vi "uRedRTP.vi"() -> ()   [LabVIEW 2019]
uses:
  <vilib>/FPGAPlugInAG/myRIO-1900/niLvFpga_Open_myRIO-1900.vi
  <vilib>/rvi/interface/common/dynamic/niFpgaDynamicAddResources.vi
  <vilib>/Utility/error.llb/Error Cluster From Error Code.vi
  <vilib>/rvi/errors/niLvFpgaAdjustHostInterfaceError.vi
  <vilib>/FPGAPlugInAG/Dynamic/niLvFpga_Close_Dynamic.vi
  <vilib>/rvi/interface/nirviOpenFPGA/nirviOpenFPGA.xnode
  FPGA Bitfiles/sec_FPGATarget2_uRedFPGA_nmZ84bOtljk.lvbitx
  uRedFPGA.vi
  <vilib>/rvi/interface/nirviReadWriteControl/nirviReadWriteControl.xnode
  <vilib>/rvi/interface/nirviCloseFPGA/nirviCloseFPGA.xnode
  NiFpgaLv.dll
  <vilib>/rvi/interface/Simulation/niFpgaSimulationCallBeginRW.vi
panel:
  out "SoCMin":bool
  out "BlocIb":bool
  out "Ib_Out":i16
  out "Vg":bool
  out "PL>PPV":bool
  out "SoC<0.8":bool
  out "mSoC":fxp<+/-,64,4>
  out "ib":fxp<+/-,64,31>
  out "Time":u32
  out "SoC":dbl(graph)
  out "Potencias":cluster{dbl, dbl, dbl}(graph)
  in  "stop":bool
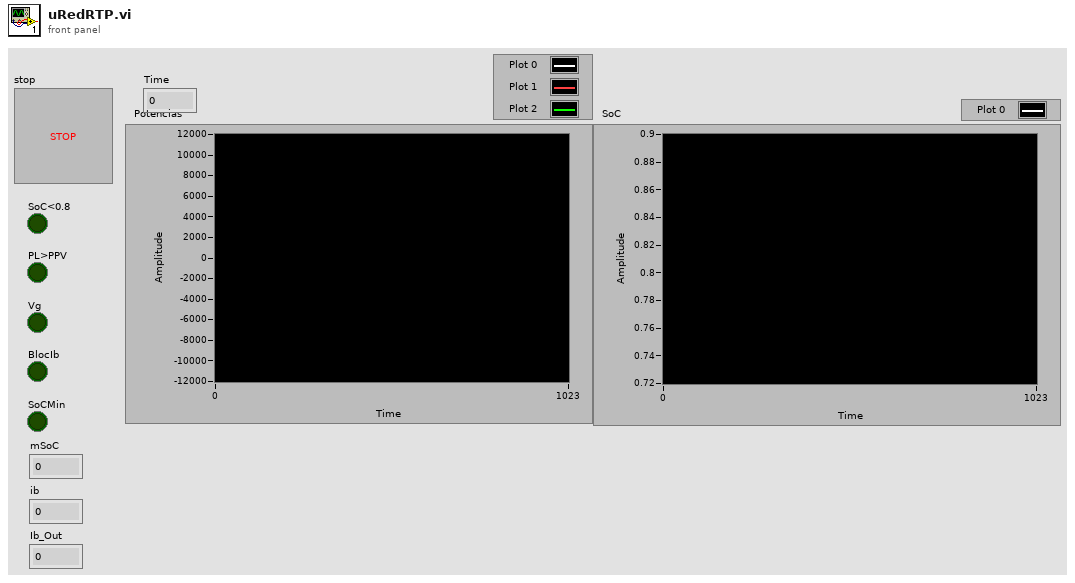
[diagram p1: front panel]
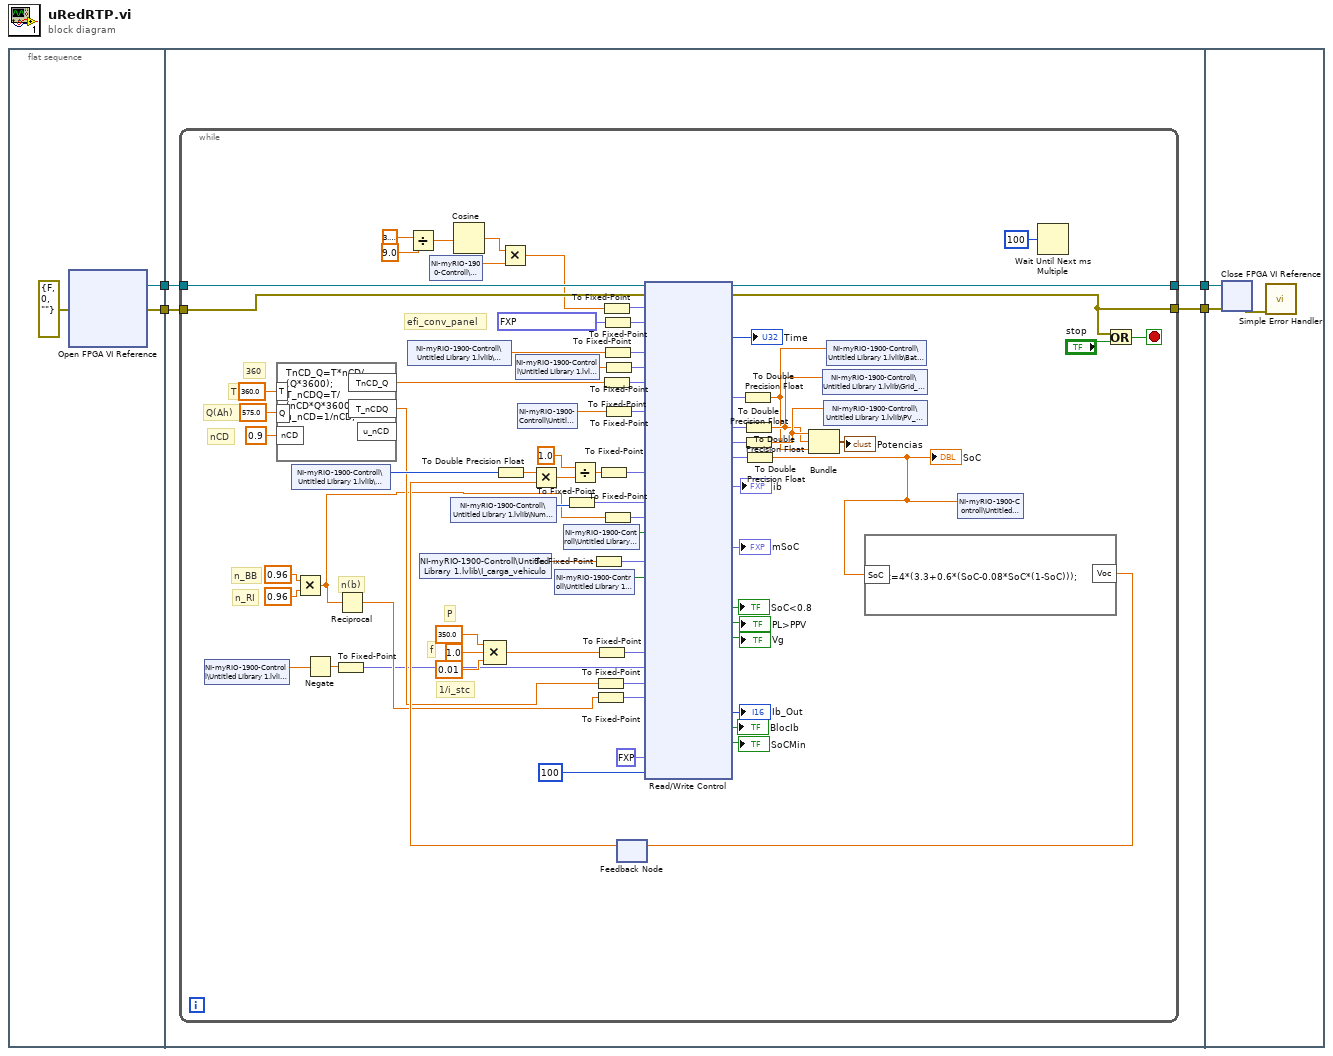
[diagram p0: block diagram]
diagram:
  n1 = flat-sequence {
    tunnel: [w7] -> w4
    tunnel: [w6] -> w3
    tunnel: w4 -> [w11]
    tunnel: w3 -> [w10]
    tunnel: [w9] -> w2
    tunnel: [w8] -> w1
    tunnel: w2 -> [w91]
    tunnel: w1 -> [w90]
    frame #0 {
      n2 = xnode "Open FPGA VI Reference"("error in"=errorcluster {"status"=FALSE, "code"=0, "source"=""}) -> ("FPGA VI Reference Out"=w7:refnum<k20>, "error out"=w6:errorcluster)  [unwired: 1 in]
    }
    frame #1 {
      n3 = while {
        tunnel: w11 -> [w86]
        tunnel: w10 -> [w85]
        tunnel: [w84] -> w9
        tunnel: [w83] -> w8
        stop <- w88 stop-if-true
        # "360"
        # "efi_conv_panel"
        # "n(b)"
        # "n_RI"
        # "n_BB"
        # "1/i_stc"
        # "f"
        # "P"
        # "nCD"
        # "T"
        # "Q(Ah)"
        n4 = shared-variable "NI-myRIO-1900-Controll\\Untitled Library 1.lvlib\\Qch_EV"() -> (w19:dbl)  [unwired: 1 in, 1 out]
        n5 = formula code="TnCD_Q=T*nCD/(Q*3600);\nT_nCDQ=T/(nCD*Q*3600);\nu_nCD=1/nCD;"("T"=360.0 ("x"), "nCD"=0.9 ("y"), "Q"=575.0) -> ("TnCD_Q"=w27:dbl, "T_nCDQ"=w25:dbl)  [unwired: 1 out]
        n6 = shared-variable "NI-myRIO-1900-Controll\\Untitled Library 1.lvlib\\Num_Bats"() -> (w45:u8)  [unwired: 1 in, 1 out]
        n7 = Multiply(x=0.96, y=0.96) -> (x*y=w20:dbl)
        n8 = Negate(x=w19) -> (-x=w18:dbl)
        n9 = To Fixed-Point(number=w18) -> (fixed-point=w17:fxp<+/-,32,16>)  [unwired: 1 in]
        n10 = Reciprocal(x=w20) -> (1/x=w22:dbl)
        n11 = Divide(x=3.141592653589793, y=9.0) -> (x/y=w51:dbl)
        n12 = shared-variable "NI-myRIO-1900-Controll\\Untitled Library 1.lvlib\\LoadPower"() -> (w42:dbl)  [unwired: 1 in, 1 out]
        n13 = shared-variable "NI-myRIO-1900-Controll\\Untitled Library 1.lvlib\\I_carga_vehiculo"() -> (w39:dbl)  [unwired: 1 in, 1 out]
        n14 = shared-variable "NI-myRIO-1900-Controll\\Untitled Library 1.lvlib\\G"() -> (w50:dbl)  [unwired: 1 in, 1 out]
        n15 = shared-variable "NI-myRIO-1900-Controll\\Untitled Library 1.lvlib\\Num_Panel"() -> (w70:u8)  [unwired: 1 in, 1 out]
        n16 = Cosine(x=w51) -> (cos(x)=w49:dbl)
        n17 = Compound Arithmetic op=MULTIPLY(350.0 ("value"), 1.0 ("value"), 0.01 ("value")) -> (w38:dbl)
        n18 = To Double Precision Float(number=w45) -> (double precision float=w46:dbl)
        n19 = Multiply(x=w49, y=w50) -> (x*y=w48:dbl)
        n20 = shared-variable "NI-myRIO-1900-Controll\\Untitled Library 1.lvlib\\SoC_ini"() -> (w69:dbl)  [unwired: 1 in, 1 out]
        n21 = shared-variable "NI-myRIO-1900-Controll\\Untitled Library 1.lvlib\\VG"() -> (w75:dbl)  [unwired: 1 in, 1 out]
        n22 = shared-variable "NI-myRIO-1900-Controll\\Untitled Library 1.lvlib\\Cargar"() -> (w41:bool)  [unwired: 1 in, 1 out]
        n23 = shared-variable "NI-myRIO-1900-Controll\\Untitled Library 1.lvlib\\InSoC"() -> (w55:bool)  [unwired: 1 in, 1 out]
        n24 = To Fixed-Point(number=w70) -> (fixed-point=w57:fxp<+,4,4>)  [unwired: 1 in]
        n25 = To Fixed-Point(number=w39) -> (fixed-point=w40:fxp<+,16,0>)  [unwired: 1 in]
        n26 = To Fixed-Point(number=w25) -> (fixed-point=w26:fxp<+,32,2>)  [unwired: 1 in]
        n27 = To Fixed-Point(number=w22) -> (fixed-point=w21:fxp<+,16,0>)  [unwired: 1 in]
        n28 = To Fixed-Point(number=w38) -> (fixed-point=w31:fxp<+,16,0>)  [unwired: 1 in]
        n29 = To Fixed-Point(number=w48) -> (fixed-point=w77:fxp<+,16,14>)  [unwired: 1 in]
        n30 = To Fixed-Point(number=w27) -> (fixed-point=w81:fxp<+,32,2>)  [unwired: 1 in]
        n31 = To Fixed-Point(number=fxp<+,16,0> 0.67999267578125) -> (fixed-point=w78:fxp<+,16,0>)  [unwired: 1 in]
        n32 = To Fixed-Point(number=w42) -> (fixed-point=w79:fxp<+,45,21>)  [unwired: 1 in]
        n33 = To Fixed-Point(number=w20) -> (fixed-point=w56:fxp<+,16,0>)  [unwired: 1 in]
        n34 = To Fixed-Point(number=w69) -> (fixed-point=w80:fxp<+,32,0>)  [unwired: 1 in]
        n35 = To Fixed-Point(number=w75) -> (fixed-point=w59:fxp<+,16,8>)  [unwired: 1 in]
        n36 = feedback #1() -> (w43:dbl)  [unwired: 1 in]
        n37 = Multiply(x=w46, y=w43) -> (x*y=w67:dbl)
        n38 = Divide(x=1.0, y=w67) -> (x/y=w66:dbl)
        n39 = To Fixed-Point(number=w66) -> (fixed-point=w58:fxp<+,16,8>)  [unwired: 1 in]
        n40 = xnode "Read/Write Control"("FPGA VI Reference In"=w86, "error in"=w85, "G"=w77, "n(p)"=w78, "PL"=w79, "SoC_in"=w80, "T*n(CD)/Q"=w81, "VG"=w59, "1/Voc"=w58, "N_Panel"=w57, "nc(b)"=w56, "P_SoC"=w55, "CC_Constant"=w40, "Cargar"=w41, "P*f/i_stc"=w31, "Q"=w17, "T/(n(CD)*Q)"=w26, "1/nc(b)"=w21, "LimSoC"=fxp<+/-,32,16> 1.0, "Time_ms"=u32 100) -> ("FPGA VI Reference Out"=w84:refnum<k20>, "error out"=w83:errorcluster, "Time(ms)"=→"Time":u32, "Pb"=w65:fxp<+/-,47,23>, "PG"=w64:fxp<+/-,47,23>, "PPV"=w63:fxp<+,45,21>, "SoC"=w62:fxp<+,32,0>, "ib"=→"ib":fxp<+/-,64,33>, "mSoC"=→"mSoC":fxp<+/-,64,4>, "SoC<0.8"=→"SoC<0.8":bool, "PL>PPV"=→"PL>PPV":bool, "Vg"=→"Vg":bool, "Ib_Out"=→"Ib_Out":i16, "BlocIb"=→"BlocIb":bool, "SoCMin"=→"SoCMin":bool)  [unwired: 1 out]
        n41 = To Double Precision Float(number=w65) -> (double precision float=w72:dbl)
        n42 = To Double Precision Float(number=w64) -> (double precision float=w73:dbl)
        n43 = To Double Precision Float(number=w63) -> (double precision float=w74:dbl)
        n44 = To Double Precision Float(number=w62) -> (double precision float=w47:dbl)
        "SoC" <- w47
        n45 = Bundle(w74, w73, w72) -> (→"Potencias":cluster{dbl, dbl, dbl})  [unwired: 1 in]
        n46 = shared-variable "NI-myRIO-1900-Controll\\Untitled Library 1.lvlib\\Grid_Power"(w73) -> ()  [unwired: 1 in, 1 out]
        n47 = shared-variable "NI-myRIO-1900-Controll\\Untitled Library 1.lvlib\\PV_POWER"(w74) -> ()  [unwired: 1 in, 1 out]
        n48 = shared-variable "NI-myRIO-1900-Controll\\Untitled Library 1.lvlib\\Bat_Power"(w72) -> ()  [unwired: 1 in, 1 out]
        n49 = formula code="Voc=4*(3.3+0.6*(SoC-0.08*SoC*(1-SoC)));"("SoC"=w47) -> ("Voc"=w44:dbl)
        n50 = feedback-in #1(w44) -> ()
        n51 = shared-variable "NI-myRIO-1900-Controll\\Untitled Library 1.lvlib\\SoC"(w47) -> ()  [unwired: 1 in, 1 out]
        n52 = Wait Until Next ms Multiple(millisecond multiple=u32 100) -> ()  [unwired: 1 out]
        n53 = Or(x=w83, y="stop") -> (x .or. y?=w88:bool)
      }
    }
    frame #2 {
      n54 = xnode "Close FPGA VI Reference"("FPGA VI Reference In"=w91, "error in"=w90) -> ("error out"=w89:errorcluster)
      n55 = call <vilib>:"Simple Error Handler.vi"("error in (no error)"=w89) -> ()  [unwired: 4 in, 5 out]
    }
  }
